vi "get_login_info.vi"(8 "error in (no error)":errorcluster, 10 "User name":string, 11 "User":string) -> (0 "error out":errorcluster, 2 "password":string, 3 "User_name":string)   [LabVIEW 2021]
panel:
  out "appended path":path
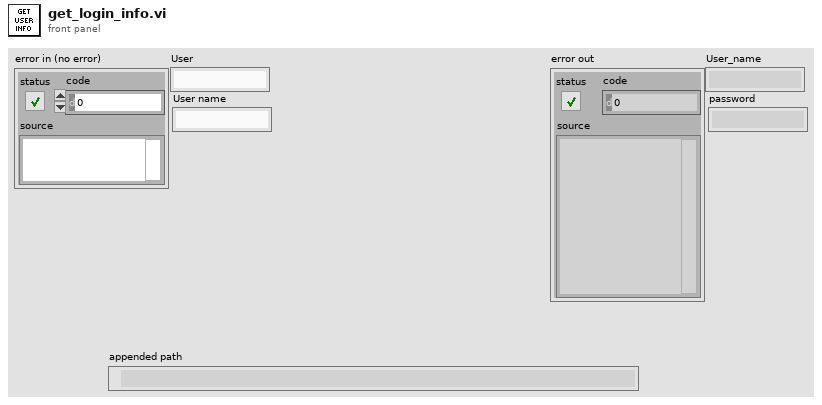
[diagram p1: front panel]
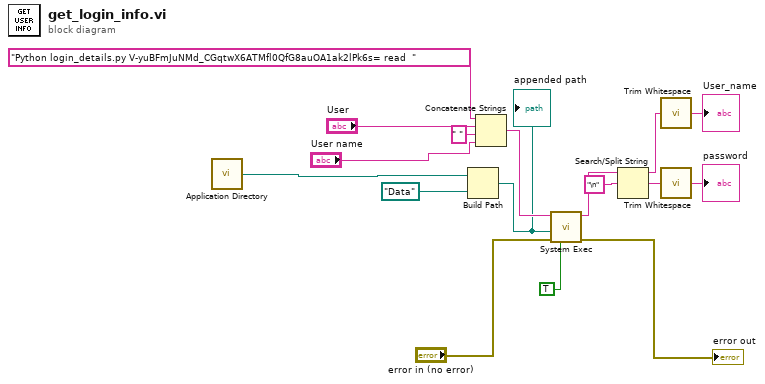
[diagram p0: block diagram]
diagram:
  n1 = call <vilib>:"Application Directory.vi"() -> ("Application Directory"=w1:path)
  n2 = Build Path(base path=w1, name or relative path=path "Data") -> (appended path=w12:path)
  "appended path" <- w12
  n3 = Concatenate Strings("Python login_details.py V-yuBFmJuNMd_CGqtwX6ATMfl0QfG8auOA1ak2lPk6s= read  ", "User", " " ("string"), "User name") -> (w14:string)
  n4 = call <vilib>:"System Exec.vi"("run minimized? (F)"=TRUE, "error in (no error)"="error in (no error)", "working directory"=w12, "command line"=w14) -> ("error out"=→"error out":errorcluster, "standard output"=w10:string)  [unwired: 4 in, 2 out]
  n5 = Search/Split String(string=w10, search string/char (-)="\n") -> (substring before match=w8:string, match + rest of string=w7:string)  [unwired: 1 in, 1 out]
  n6 = call <vilib>:"Trim Whitespace.vi"("string"=w8) -> ("trimmed string"=→"User_name":string)  [unwired: 1 in]
  n7 = call <vilib>:"Trim Whitespace.vi"("string"=w7) -> ("trimmed string"=→"password":string)  [unwired: 1 in]
